vi "Periodic Tasks.vi"(8 "error in":errorcluster) -> ()   [LabVIEW 2016]
doc: "This VI runs in parallel to other tasks. It can contain as many user-defined periodic loops as you need. These can carry out PID or other sorts of timed response."
uses:
  <vilib>/Rock Robotics/WPI/DriverStation/WPI_DriverStationRobotMode2.ctl
  <vilib>/Rock Robotics/WPI/Utilities/WPI_GetSetVariantRefNum.vi
  Robot Global Data.vi
  AutoLeftDrive.vi
  AutoRightDrive.vi
  <vilib>/Rock Robotics/Network Tables/NT Write Number.vi
  <vilib>/Rock Robotics/WPI/Ultrasonic/WPI_SonarSRF04DigitalRefNum Registry Get.vi
  <vilib>/Rock Robotics/WPI/Ultrasonic/WPI_SonarSRF04DigitalGetRange.vi
  Target x Location.vi
  AutoModEnable.vi
  AutoProceed.vi
  AutoMod.vi
panel:
  out "Auto Mod Enable":bool
  out "Target x Location contr":dbl
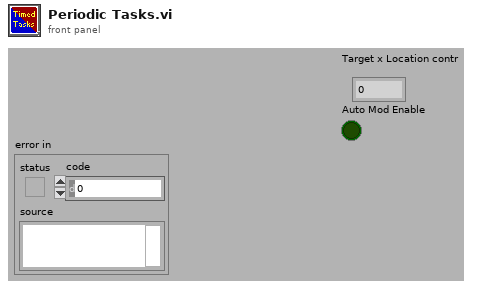
[diagram p1: front panel]
types:
  T1 = typedef "WPI_JoystickDevRef.ctl" = cluster{"Device":T2}
  T2 = typedef "WPI_JoystickDeviceEnum.ctl" = enum16{"USB 0", "USB 1", "USB 2", "USB 3", "USB 4", "USB 5"}
  T3 = typedef "WPI_RobotDriveDevRef.ctl" = cluster{"DevStatus":errorcluster, "Motors[]":T4[], "Square Inputs":bool, "Max Output":dbl}
  T4 = typedef "WPI_MotorControlDeviceRef.ctl" = cluster{"DeviceStatus":errorcluster, "Type":T5, "PWM":cluster{"PWM Channel":T6, "DeadBand":T7}, "CAN":cluster{"Device Number":u8, "SetOutput VI Ref":variant, "GetOutput VI Ref":variant, "Enable VI Ref":variant, "Disable VI Ref":variant, "Data":variant}, "Invert":bool}
  T5 = typedef "WPI_MotorControlType.ctl" = enum16{"PWM", "CAN"}
  T6 = typedef "FPGA_DIOPWMChannel.ctl" = enum8{"PWM 0", "PWM 1", "PWM 2", "PWM 3", "PWM 4", "PWM 5", "PWM 6", "PWM 7", "PWM 8", "PWM 9", "PWM MXP 0", "PWM MXP 1", "PWM MXP 2", "PWM MXP 3", "PWM MXP 4", "PWM MXP 5", "PWM MXP 6", "PWM MXP 7", "PWM MXP 8", "PWM MXP 9", "Invalid"}
  T7 = typedef "WPI_PWMDeadband.ctl" = cluster{"Name":string, "maxPositivePwm":i32, "minPositivePwm":i32, "centerPwm":i32, "maxNegativePwm":i32, "minNegativePwm":i32, "angularRange":u16}
  T8 = cluster{"JoystickDevRef":T1, "RobotDriveDevRef":T3}
  T9 = typedef "WPI_DriverStationRobotMode2.ctl" = enum16{"Autonomous Disabled", "Autonomous Enabled", "Teleop Disabled", "Teleop Enabled", "Disconnected", "Finish", "Test Disabled", "Test Enabled", "Emergency Stopped"}
  T10 = typedef "WPI_GyroDevRef.ctl" = cluster{"DevStatus":errorcluster, "Analog Channel":T11, "Offset":dbl, "Gain (VoltsPerDegree/Second)":dbl, "Gyro Type":enum16{"Analog", "XRS450"}, "Handle":i32, "SPI Bus":T12, "Device Found":bool, "Sample Rate":dbl, "Calibrate On Open":bool}
  T11 = typedef "FPGA_AIChannel.ctl" = enum8{"AI 0", "AI 1", "AI 2", "AI 3", "AI MXP 0", "AI MXP 1", "AI MXP 2", "AI MXP 3", "Invalid"}
  T12 = typedef "spi_bus.ctl" = enum16{"SPI On-Board, CS0", "SPI On-Board, CS1", "SPI On-Board, CS2", "SPI On-Board, CS3", "SPI MXP", "Invalid"}
  T13 = typedef "WPI_UltrasonicDeviceRef.ctl" = cluster{"DevStatus":errorcluster, "Ping Channel":T14, "Echo Channel":T14, "CntIndex":T15}
  T14 = typedef "FPGA_DIOChannel.ctl" = enum8{"DIO 0", "DIO 1", "DIO 2", "DIO 3", "DIO 4", "DIO 5", "DIO 6", "DIO 7", "DIO 8", "DIO 9", "DIO MXP 0", "DIO MXP 1", "DIO MXP 2", "DIO MXP 3", "DIO MXP 4", "DIO MXP 5", "DIO MXP 6", "DIO MXP 7", "DIO MXP 8", "DIO MXP 9", "DIO MXP 10", "DIO MXP 11", "DIO MXP 12", "DIO MXP 13", "DIO MXP 14", "DIO MXP 15", "SPI Port CS1", "SPI Port CS2", "SPI Port CS3", "SPI Port MISO", "SPI Port MOSI", "Invalid"}
  T15 = typedef "FPGA_CounterCtrSystemIndex.ctl" = enum8{"Ctr 0", "Ctr 1", "Ctr 2", "Ctr 3", "Ctr 4", "Ctr 5", "Ctr 6", "Ctr 7", "Invalid"}
  T16 = typedef "WPI_EncoderDevRef.ctl" = cluster{"DevStatus":errorcluster, "EncoderIndex":T17, "CounterIndex":T15, "DistancePerCount":dbl, "Decoding Type":T18}
  T17 = typedef "FPGA_EncoderIdx.ctl" = enum8{"Enc 0", "Enc 1", "Enc 2", "Enc 3", "Enc 4", "Enc 5", "Enc 6", "Enc 7", "Invalid"}
  T18 = typedef "WPI_EncoderType.ctl" = enum16{"1x", "2x", "4x"}
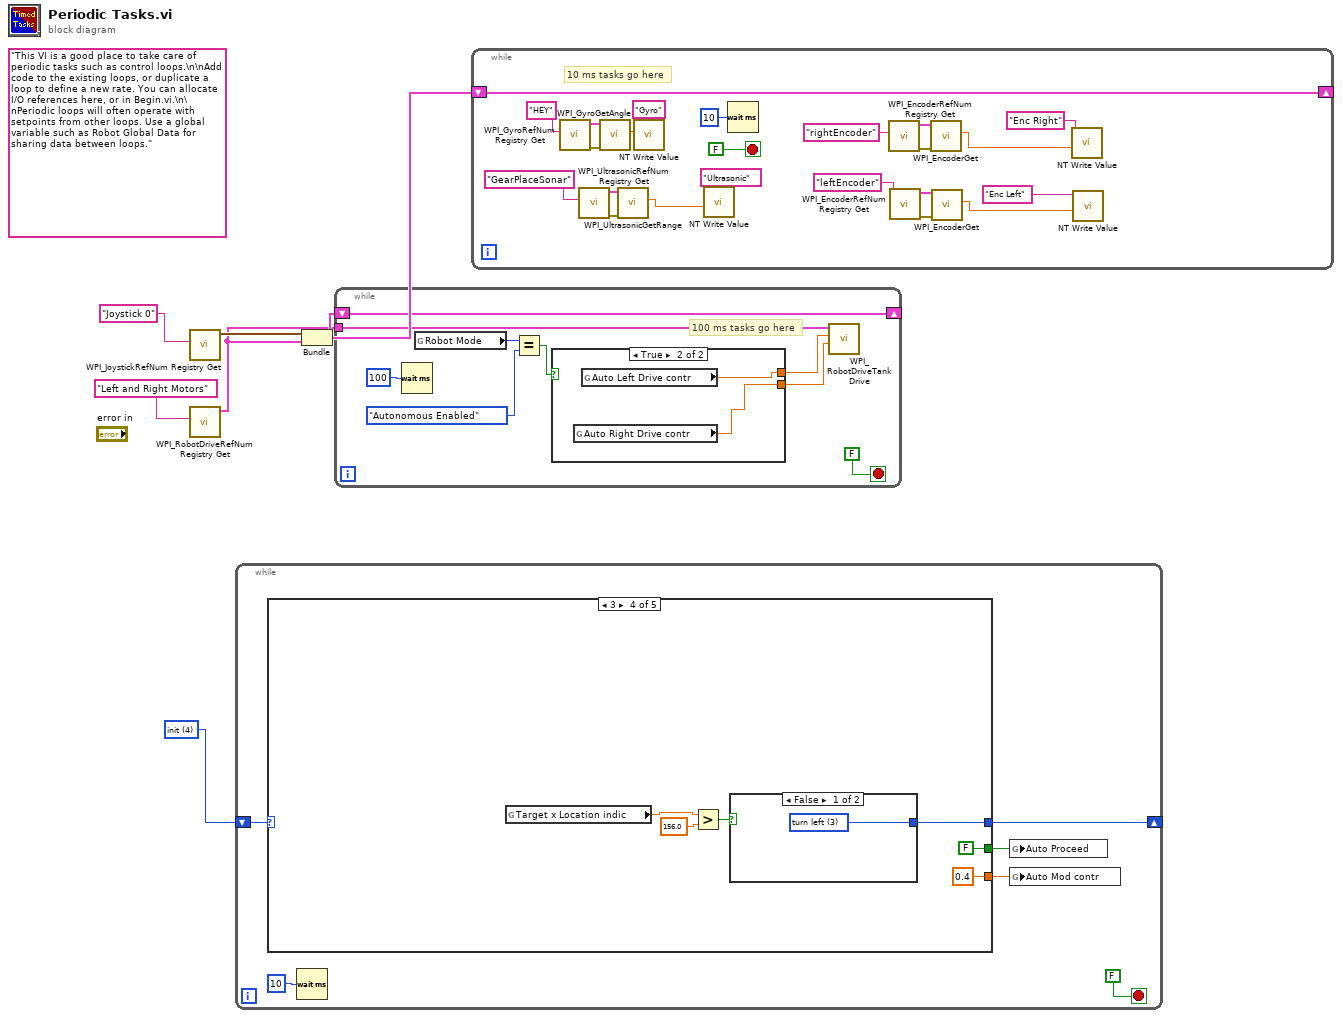
[diagram p0: block diagram]
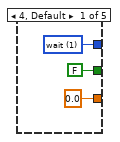
[diagram p2: hidden frame]
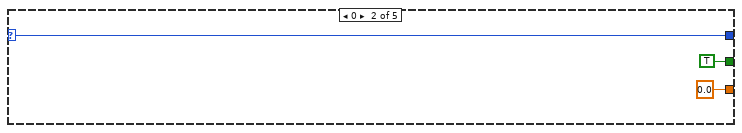
[diagram p3: hidden frame]
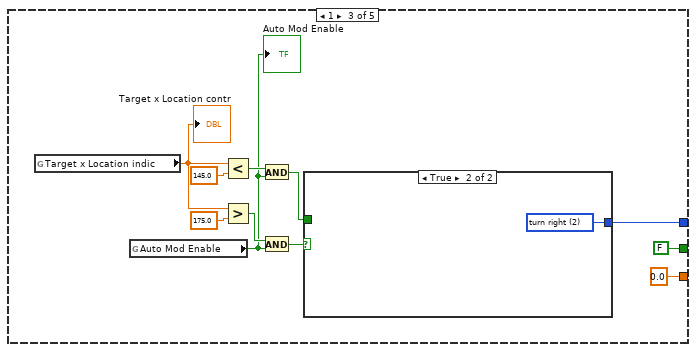
[diagram p4: hidden frame]
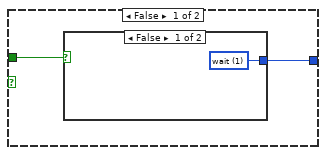
[diagram p5: hidden frame]
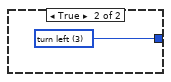
[diagram p6: hidden frame]
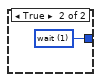
[diagram p7: hidden frame]
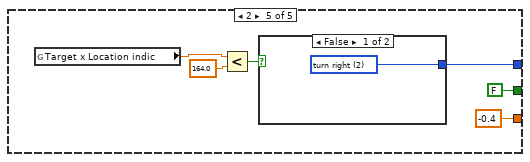
[diagram p8: hidden frame]
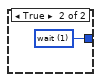
[diagram p9: hidden frame]
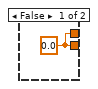
[diagram p10: hidden frame]
diagram:
  w2 = u16 4 items=["stop", "wait", "turn right", "turn left", "init"]
  (unwired) "This VI is a good place to take care of periodic tasks such as control loops.\n\nAdd code to the existing loops, or duplicate a loop to define a new rate. You can allocate I/O references here, or in Begin.vi.\n\nPeriodic loops will often operate with setpoints from other loops. Use a global variable such as Robot Global Data for sharing data between loops."
  n1 = call <vilib>:"WPI_JoystickRefNum Registry Get.vi"("refnum name"="Joystick 0") -> ("JoystickDevRef"=w4:T1)  [unwired: 1 in, 9 out]
  n2 = call <vilib>:"WPI_RobotDriveRefNum Registry Get.vi"("refnum name"="Left and Right Motors") -> ("RobotDriveDevRef"=w1:T3)  [unwired: 1 in, 9 out]
  n3 = while {
    shift-right: [w8] -> _
    shift-left: w2 -> [w7]
    stop <- FALSE stop-if-true
    n4 = case shown="3" w7 {
      selector: w7 -> [_ w16 _ _ _]
      tunnel: [0.0 0.0 0.0 0.4 -0.4] -> w10
      tunnel: [FALSE TRUE FALSE FALSE FALSE] -> w9
      tunnel: [w13 w16 w21 w37 w45] -> w8
      frame 4, Default {
        w13 = u16 1 items=["stop", "wait", "turn right", "turn left", "init"]
      }
      frame 0 {
      }
      frame 1 {
        n5 = global read "Target x Location.vi" "Target x Location indic"() -> (w28:dbl)
        "Target x Location contr" <- w28
        n6 = global read "AutoModEnable.vi" "Auto Mod Enable"() -> (w24:bool)
        "Auto Mod Enable" <- w24
        n7 = Less?(x=w28, y=145.0) -> (x < y?=w25:bool)
        n8 = Greater?(x=w28, y=175.0) -> (0:w26:bool)
        n9 = And(x=w25, y=w24) -> (x .and. y?=w22:bool)
        n10 = And(x=w26, y=w24) -> (x .and. y?=w23:bool)
        n11 = case shown="True" w23 {
          tunnel: w22 -> [w31 _]
          tunnel: [w30 w34] -> w21
          frame False {
            n12 = case shown="False" w31 {
              tunnel: [w32 w33] -> w30
              frame False {
                w32 = u16 1 items=["stop", "wait", "turn right", "turn left", "init"]
              }
              frame True {
                w33 = u16 3 items=["stop", "wait", "turn right", "turn left", "init"]
              }
            }
          }
          frame True {
            w34 = u16 2 items=["stop", "wait", "turn right", "turn left", "init"]
          }
        }
      }
      frame 3 {
        n13 = global read "Target x Location.vi" "Target x Location indic"() -> (w40:dbl)
        n14 = Greater?(x=w40, y=156.0) -> (0:w38:bool)
        n15 = case shown="False" w38 {
          tunnel: [w41 w42] -> w37
          frame False {
            w41 = u16 3 items=["stop", "wait", "turn right", "turn left", "init"]
          }
          frame True {
            w42 = u16 1 items=["stop", "wait", "turn right", "turn left", "init"]
          }
        }
      }
      frame 2 {
        n16 = global read "Target x Location.vi" "Target x Location indic"() -> (w48:dbl)
        n17 = Less?(x=w48, y=164.0) -> (x < y?=w46:bool)
        n18 = case shown="False" w46 {
          tunnel: [w49 w50] -> w45
          frame False {
            w49 = u16 2 items=["stop", "wait", "turn right", "turn left", "init"]
          }
          frame True {
            w50 = u16 1 items=["stop", "wait", "turn right", "turn left", "init"]
          }
        }
      }
    }
    n19 = Wait (ms)(milliseconds to wait=u32 10) -> ()  [unwired: 1 out]
    n20 = global write "AutoProceed.vi" "Auto Proceed"(w9) -> ()
    n21 = global write "AutoMod.vi" "Auto Mod contr"(w10) -> ()
  }
  n22 = Bundle("JoystickDevRef"=w4, "RobotDriveDevRef"=w1) -> (w3:T8)  [unwired: 1 out]
  n23 = while {
    shift-right: [w57] -> _
    shift-left: w3 -> [w57]
    tunnel: w1 -> [w51]
    stop <- FALSE stop-if-true
    # "100 ms tasks go here"
    n24 = Wait (ms)(milliseconds to wait=u32 100) -> ()  [unwired: 1 out]
    n25 = global read "Robot Global Data.vi" "Robot Mode"() -> (w54:T9)
    n26 = Equal?(x=w54, y=WPI_DriverStationRobotMode2."Autonomous Enabled" ("Robot Mode")) -> (x = y?=w56:bool)
    n27 = case shown="True" w56 {
      tunnel: [w60 w61] -> w53
      tunnel: [w60 w62] -> w52
      frame False {
        w60 = 0.0
      }
      frame True {
        n28 = global read "AutoRightDrive.vi" "Auto Right Drive contr"() -> (w62:dbl)
        n29 = global read "AutoLeftDrive.vi" "Auto Left Drive contr"() -> (w61:dbl)
      }
    }
    n30 = call <vilib>:"WPI_RobotDriveTankDrive.vi"("Right axis value"=w52, "Left axis value"=w53, "RobotDriveDevRef"=w51) -> ()  [unwired: 6 in, 3 out]
  }
  n31 = while {
    shift-right: [w83] -> _
    shift-left: w3 -> [w83]
    stop <- FALSE stop-if-true
    # "10 ms tasks go here"
    n32 = call <vilib>:"WPI_GyroRefNum Registry Get.vi"("refnum name"="HEY") -> ("error out"=w74:errorcluster, "GyroDevRef"=w75:T10)  [unwired: 9 in]
    n33 = call-poly <vilib>:"WPI_UltrasonicRefNum Registry Get.vi"("refnum name"="GearPlaceSonar") -> ("error out"=w78:errorcluster, "SonarSRF04DevRef"=w79:T13)  [unwired: 9 in]
    n34 = call <vilib>:"WPI_GyroGetAngle.vi"("error in"=w74, "GyroDevRef"=w75) -> ("Angle"=w77:dbl)  [unwired: 5 in, 4 out]
    n35 = call-poly <vilib>:"WPI_UltrasonicGetRange.vi"("error in (no error)"=w78, "SonarSRF04DevRef"=w79) -> ("Distance"=w80:dbl)  [unwired: 7 in, 2 out]
    n36 = call-poly <vilib>:"NT Write Value.vi"("Numeric"=w77, "Name"="Gyro") -> ()  [unwired: 9 in, 1 out]
    n37 = call-poly <vilib>:"NT Write Value.vi"("Numeric"=w80, "Name"="Ultrasonic") -> ()  [unwired: 9 in, 1 out]
    n38 = Wait (ms)(milliseconds to wait=u32 10) -> ()  [unwired: 1 out]
    n39 = call <vilib>:"WPI_EncoderRefNum Registry Get.vi"("refnum name"="rightEncoder") -> ("error out"=w68:errorcluster, "EncoderDevRef"=w67:T16)  [unwired: 9 in]
    n40 = call <vilib>:"WPI_EncoderRefNum Registry Get.vi"("refnum name"="leftEncoder") -> ("error out"=w66:errorcluster, "EncoderDevRef"=w65:T16)  [unwired: 9 in]
    n41 = call <vilib>:"WPI_EncoderGet.vi"("error in (no error)"=w68, "EncoderDevRef"=w67) -> ("Distance"=w64:dbl)  [unwired: 4 in, 5 out]
    n42 = call <vilib>:"WPI_EncoderGet.vi"("error in (no error)"=w66, "EncoderDevRef"=w65) -> ("Distance"=w63:dbl)  [unwired: 4 in, 5 out]
    n43 = call-poly <vilib>:"NT Write Value.vi"("Numeric"=w64, "Name"="Enc Right") -> ()  [unwired: 9 in, 1 out]
    n44 = call-poly <vilib>:"NT Write Value.vi"("Numeric"=w63, "Name"="Enc Left") -> ()  [unwired: 9 in, 1 out]
  }
